vi "Test Non-JSON Request Gets Parse Error.vi"(8 "error in (no error)":errorcluster) -> (0 "error out":errorcluster)   [LabVIEW 2019, in "RemoteControl.ZMQ.Tests.lvclass"]
uses:
  RemoteControl.ZMQ.Tests.lvclass
  <vilib>/addons/zeromq/socket_type.ctl
  <vilib>/addons/_JKI Toolkits/Caraya/classes/Assert/Assert True.vi
  <vilib>/addons/_JKI Toolkits/Caraya/classes/Assert/Assert.lvclass
  <vilib>/addons/_JKI Toolkits/Caraya/classes/Test/Test.lvclass
  <vilib>/addons/zeromq/zmq_context.lvclass
  <vilib>/addons/zeromq/zeromq.lvlib
  <vilib>/addons/zeromq/zmq_socket.lvclass
  <vilib>/PRIrvin/JSON-RPC/JSON-RPC.lvlib
panel:
  out "data":string
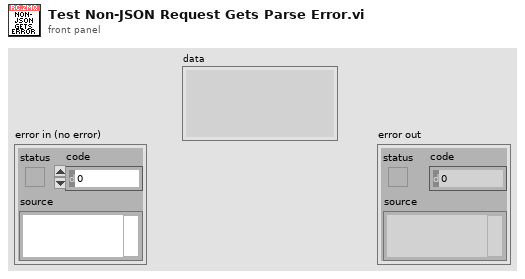
[diagram p1: front panel]
types:
  T1 = typedef "zeromq.lvlib/socket_type.ctl" = enum8{"ZMQ_PAIR", "ZMQ_PUB", "ZMQ_SUB", "ZMQ_REQ", "ZMQ_REP", "ZMQ_DEALER", "ZMQ_ROUTER", "ZMQ_PULL", "ZMQ_PUSH", "ZMQ_XPUB", "ZMQ_XSUB", "ZMQ_STREAM", "ZMQ_SERVER", "ZMQ_CLIENT", "ZMQ_RADIO", "ZMQ_DISH", "ZMQ_GATHER", "ZMQ_SCATTER", "ZMQ_DGRAM"}
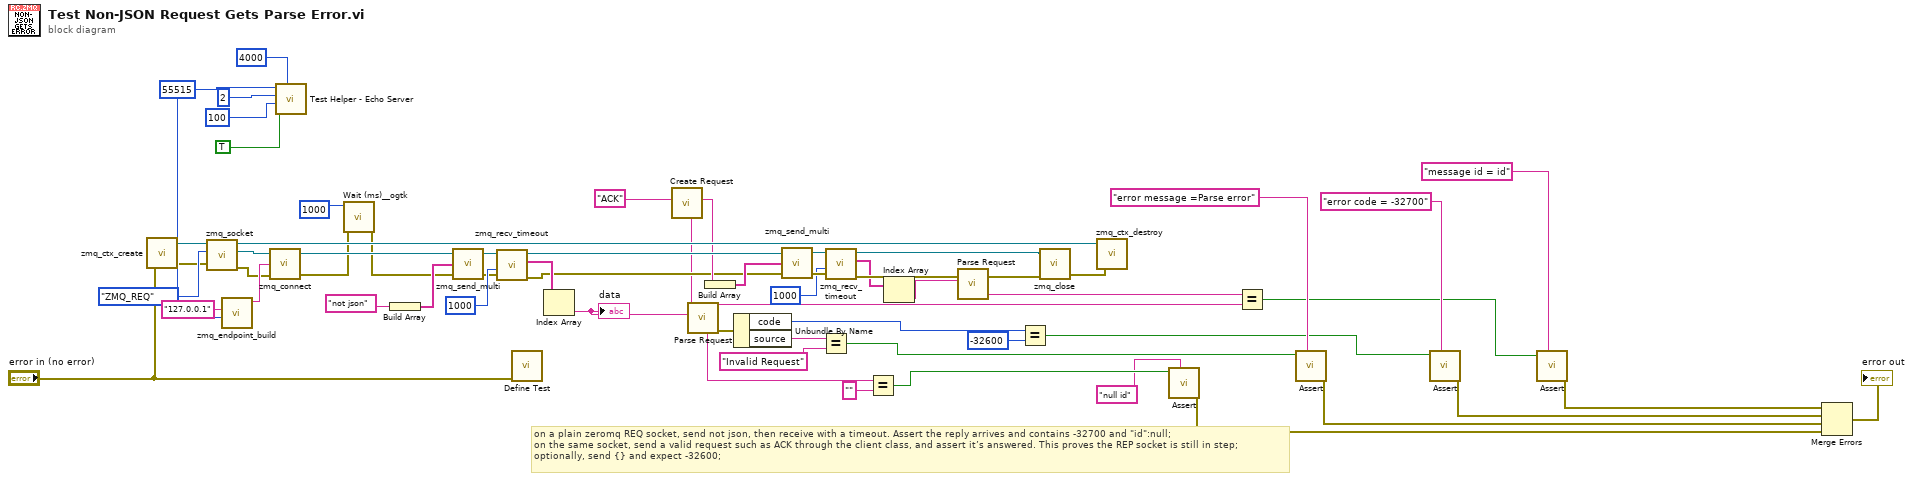
[diagram p0: block diagram]
diagram:
  w51 = u16 55515 ("Port")
  # "on a plain zeromq REQ socket, send not json, then receive with a timeout. Assert the reply arrives and contains -32700 and \"id\":null;\non the same socket, send a valid request such as ACK through the client class, and assert it’s answered. This proves the REP socket is still in step;\noptionally, send {} and expect -32600;"
  n1 = call <vilib>:"zmq_ctx_create.vi"("error in"="error in (no error)") -> ("error out"=w45:errorcluster, "context out"=w54:refnum<class "zmq_context.lvclass">)  [unwired: 3 in]
  n2 = call <vilib>:"zmq_socket.vi"("error in"=w45, "socket type"=socket_type."ZMQ_REQ", "context in"=w54) -> ("error out"=w37:errorcluster, "socket out"=w50:refnum<class "zmq_socket.lvclass">, "context out"=w47:refnum<class "zmq_context.lvclass">)  [unwired: 2 in]
  n3 = call <vilib>:"zmq_endpoint_build.vi"("port"=w51, "address"="127.0.0.1") -> ("endpoint"=w52:string)  [unwired: 3 in, 2 out]
  n4 = call <vilib>:"zmq_connect.vi"("error in"=w37, "endpoint"=w52, "socket in"=w50) -> ("error out"=w3:errorcluster, "socket out"=w42:refnum<class "zmq_socket.lvclass">)  [unwired: 1 in]
  n5 = call "Test Helper - Echo Server.vi"("idle timout"=u32 4000, "Answer?"=TRUE, "reply delay (ms)"=u32 100, "number of messages"=2, "port"=w51) -> ()  [unwired: 5 in, 2 out]
  n6 = call <userlib>:"Wait (ms)__ogtk.vi"("error in (no error)"=w3, "milliseconds to wait"=u32 1000 ("timeout (ms)")) -> ("error out"=w2:errorcluster)  [unwired: 8 in, 1 out]
  n7 = Build Array("not json" ("data")) -> (w38:string[])
  n8 = call <vilib>:"zmq_send_multi.vi"("error in"=w2, "parts"=w38, "socket in"=w42) -> ("error out"=w40:errorcluster, "socket out"=w41:refnum<class "zmq_socket.lvclass">)  [unwired: 1 in]
  n9 = call <vilib>:"zmq_recv_timeout.vi"("error in"=w40, "timeout (ms)"=u32 1000, "socket in"=w41) -> ("error out"=w19:errorcluster, "parts"=w48:string[], "socket out"=w26:refnum<class "zmq_socket.lvclass">)  [unwired: 1 in, 1 out]
  n10 = call <vilib>:"Define Test.vi"("error in (no error)"="error in (no error)") -> ()  [unwired: 9 in, 2 out]
  n11 = Index Array(array=w48) -> (element=w36:string)  [unwired: 1 in]
  "data" <- w36
  n12 = call <vilib>:"Create Request.vi"("method"="ACK" ("data")) -> ("<JSON> Requests"=w21:string, "IDs"=w12:string)  [unwired: 8 in, 1 out]
  n13 = call <vilib>:"Parse Request.vi"("<JSON> Requests"=w36) -> ("error out"=w35:errorcluster, "IDs"=w8:string)  [unwired: 7 in, 2 out]
  n14 = Build Array(w21) -> (w20:string[])
  n15 = Unbundle By Name(w35) -> ("code"=w31:i32, "source"=w34:string)
  n16 = call <vilib>:"zmq_send_multi.vi"("error in"=w19, "parts"=w20, "socket in"=w26) -> ("error out"=w28:errorcluster, "socket out"=w25:refnum<class "zmq_socket.lvclass">)  [unwired: 1 in]
  n17 = Equal?(x=w34, y="Invalid Request") -> (x = y?=w32:bool)
  n18 = call <vilib>:"zmq_recv_timeout.vi"("error in"=w28, "timeout (ms)"=u32 1000, "socket in"=w25) -> ("error out"=w23:errorcluster, "parts"=w15:string[], "socket out"=w24:refnum<class "zmq_socket.lvclass">)  [unwired: 1 in, 1 out]
  n19 = Equal?(x=w8, y="") -> (x = y?=w6:bool)
  n20 = Index Array(array=w15) -> (element=w14:string)  [unwired: 1 in]
  n21 = call <vilib>:"Parse Request.vi"("<JSON> Requests"=w14) -> ("IDs"=w13:string)  [unwired: 7 in, 3 out]
  n22 = Equal?(x=w31, y=-32600) -> (x = y?=w29:bool)
  n23 = call <vilib>:"zmq_close.vi"("error in"=w23, "socket"=w24) -> ("error out"=w46:errorcluster)  [unwired: 3 in]
  n24 = call <vilib>:"zmq_ctx_destroy.vi"("error in"=w46, "context in"=w47) -> ()  [unwired: 3 in, 1 out]
  n25 = call-poly <vilib>:"Assert.vi"("Label"="null id", "True?"=w6) -> ("error out"=w4:errorcluster)  [unwired: 8 in, 1 out]
  n26 = Equal?(x=w13, y=w12) -> (x = y?=w11:bool)
  n27 = call-poly <vilib>:"Assert.vi"("Label"="error message =Parse error", "True?"=w32) -> ("error out"=w17:errorcluster)  [unwired: 8 in, 1 out]
  n28 = call-poly <vilib>:"Assert.vi"("Label"="error code = -32700", "True?"=w29) -> ("error out"=w18:errorcluster)  [unwired: 8 in, 1 out]
  n29 = call-poly <vilib>:"Assert.vi"("Label"="message id = id", "True?"=w11) -> ("error out"=w10:errorcluster)  [unwired: 8 in, 1 out]
  n30 = Merge Errors(w10, w18, w17, w4) -> (→"error out":errorcluster)
